vi "W12_History_test.vi"() -> ()   [LabVIEW 2026]
doc: "Use this template to build a VI to use as a subVI."
panel:
  out "history (last)":dbl[](array[numeric])
  out "length (each reading)":i32[](array[numeric])
  in  "N (keep the last N)":i32
  in  "values":dbl[](array[numeric])
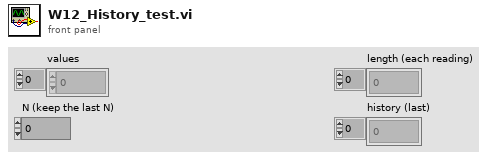
[diagram p1: front panel]
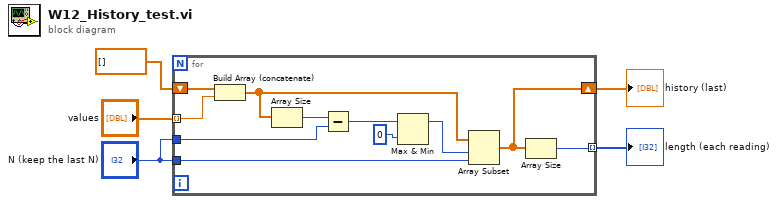
[diagram p0: block diagram]
diagram:
  n1 = for {
    shift-right: [w7] -> w1
    shift-left: dbl[] [] -> [w16]
    tunnel: "values" -> [w15] mode=indexing
    tunnel: "N (keep the last N)" -> [w12]
    tunnel: "N (keep the last N)" -> [w8]
    tunnel: [w6] -> w2 mode=indexing
    n2 = Build Array (concatenate)(w16, w15) -> (w14:dbl[])
    n3 = Array Size(array=w14) -> (size(s)=w13:i32)
    n4 = Subtract(x=w13, y=w12) -> (x-y=w11:i32)
    n5 = Max & Min(x=w11, y=0) -> (max(x,y)=w9:i32)  [unwired: 1 out]
    n6 = Array Subset(array=w14, index=w9, length=w8) -> (w7:dbl[])
    n7 = Array Size(array=w7) -> (size(s)=w6:i32)
  }
  "length (each reading)" <- w2
  "history (last)" <- w1
